vi "ClassAttributes_GetClassAttributes_6x8x6.vi"(0 "reference in":refnum<class>, 1 "OnlyGetDvrReference(False)":bool, 5 "error in":errorcluster) -> (14 "reference out":refnum<class>, 15 "Class attribute":T1, 17 "Class attribute Reference":refnum<data-value>, 19 "error out":errorcluster)   [LabVIEW 2020]
doc: "Returns the class attributes of this class or a sub class. If reference is wired, the class attributes of the class (or sub class) will be returned else the class attributes will default to this class.\n\nIf the data is currently locked for modification, 'Attributes locked?' will return TRUE. If reference is wired, the class attributes of this class (or sub class) will be returned else the class attributes of this class."
uses:
  ClassAttributes_ClassAttributes.ctl
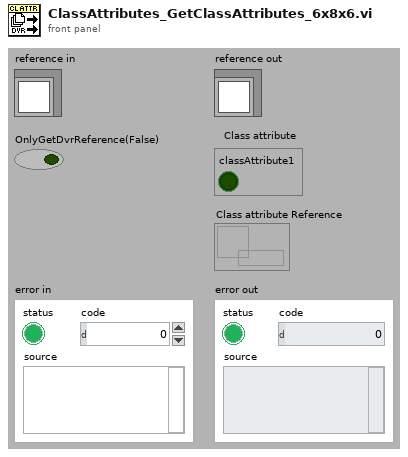
[diagram p1: front panel]
types:
  T1 = typedef "ClassAttributes_ClassAttributes.ctl" = cluster{"classAttribute1":bool}
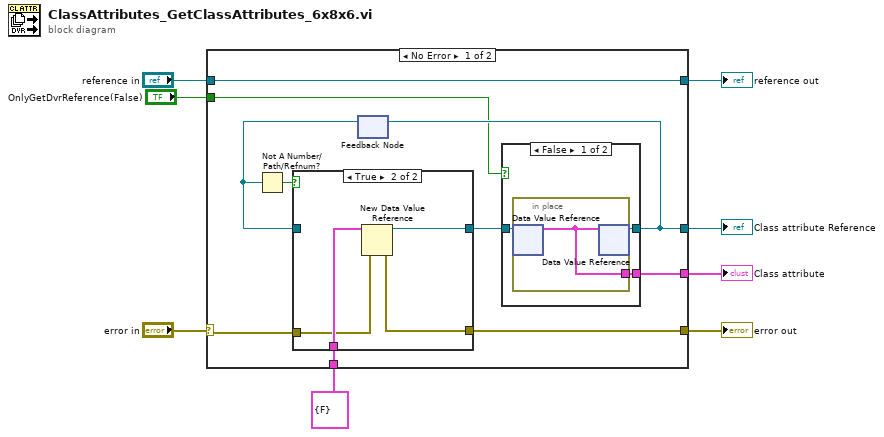
[diagram p0: block diagram]
diagram:
  n1 = case shown="No Error" "error in" {
    selector: "error in" -> [w16 w30]
    tunnel: [w18 w31] -> w8
    tunnel: [w15 w30] -> w7
    tunnel: "reference in" -> [w18 w31]
    tunnel: T1 {"classAttribute1"=FALSE} ("Class attributes") -> [w17 _]
    tunnel: [w13 _] -> w3
    tunnel: [w14 _] -> w2
    tunnel: "OnlyGetDvrReference(False)" -> [w9 _]
    frame No Error {
      n2 = feedback #1() -> (w10:refnum<data-value>)  [unwired: 1 in]
      n3 = Not A Number/Path/Refnum?(number/path/refnum=w10) -> (NaN/Path/Refnum?=w11:bool)
      n4 = case shown="True" w11 {
        tunnel: w17 -> [_ w24]
        tunnel: w16 -> [w19 w22]
        tunnel: [w19 w21] -> w15
        tunnel: [w20 w23] -> w12
        tunnel: w10 -> [w20 _]
        frame False {
        }
        frame True {
          n5 = New Data Value Reference(data value=w24, error in=w22) -> (data value reference=w23:refnum<data-value>, error out=w21:errorcluster)
        }
      }
      n6 = case shown="False" w9 {
        tunnel: [w27 _] -> w14
        tunnel: [w26 w29] -> w13
        tunnel: w12 -> [w25 w29]
        frame False {
          n7 = in-place {
            in-place-border: [w28] -> w27
            n8 = in-place-dvr #2(w25) -> (w28:T1)  [unwired: 1 out]
            n9 = in-place-dvr #2(w28) -> (w26:refnum<data-value>)  [unwired: 1 out]
          }
        }
        frame True {
        }
      }
      n10 = feedback-in #1(w13) -> ()
    }
    frame Error {
    }
  }
  "error out" <- w7
  "reference out" <- w8
  "Class attribute" <- w2
  "Class attribute Reference" <- w3
